vi "test Import Configuration File Max Channels.vi"(8 "error in":errorcluster, 11 "TestCase in":refnum<class "Import.lvclass">) -> (0 "error out":errorcluster, 3 "TestCase out":refnum<class "Import.lvclass">)   [LabVIEW 2020, in "Import.lvclass"]
uses:
  Import.lvclass
  Import.lvclass/Import.ctl
  C:/Program Files/National Instruments/LabVIEW 2026/vi.lib/addons/_JKI Toolkits/VI Tester/TestCase.llb/TestCase.lvclass
  C:/git/fmussi_niveristand-aim-arinc429-custom-device/Source/Custom Device Support/Tests/Unit/Import/Import.lvclass
  <vilib>/addons/_JKI Toolkits/VI Tester/TestCase.llb/TestCase.lvclass
  Import/ARINC 429 Import.lvlib
  <userlib>/_OpenG.lib/appcontrol/appcontrol.llb/openg_application_control.lvlib
  <vilib>/NI/VeriStand Custom Device Testing Tools/VeriStandTestUtilities/VeriStandTestUtilities.lvlib
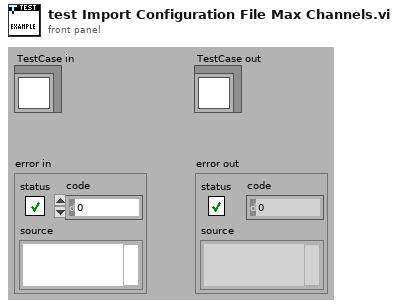
[diagram p1: front panel]
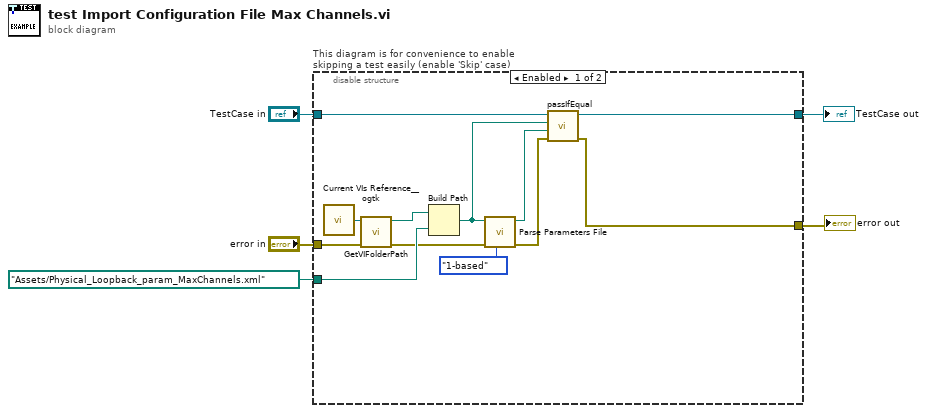
[diagram p0: block diagram]
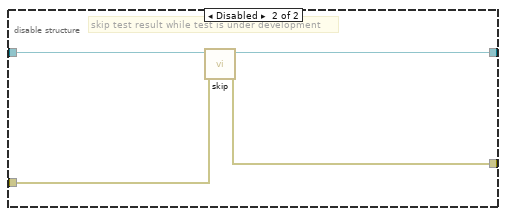
[diagram p2: hidden frame]
diagram:
  n1 = disable-structure "This diagram is for convenience to enable skipping a test easily (enable 'Skip' case)" shown="Enabled" {
    disable-tunnel: "TestCase in" -> [w17 w21]
    disable-tunnel: [w9 w19] -> w2
    disable-tunnel: [w10 w20] -> w4
    disable-tunnel: "error in" -> [w14 w18]
    disable-tunnel: path "Assets/Physical_Loopback_param_MaxChannels.xml" ("Absolute or Relative Path") -> [w13 _]
    frame Enabled {
      n2 = call <userlib>:"Current VIs Reference__ogtk.vi"() -> ("Current VI's reference"=w16:refnum<vi>)  [unwired: 5 in]
      n3 = call <vilib>:"GetVIFolderPath.vi"("error in (no error)"=w14, "VI Reference in"=w16) -> ("error out"=w11:errorcluster, "VI Folder Path out"=w15:path)  [unwired: 8 in]
      n4 = Build Path(base path=w15, name or relative path=w13) -> (appended path=w12:path)
      n5 = call "Parse Parameters File.vi"("ch indexing (0-based)"=enum16{"0-based", "1-based"}."1-based", "error in"=w11, "path to XML document"=w12) -> ("error out"=w8:errorcluster, "path to XML document out"=w7:path)  [unwired: 6 in, 1 out]
      n6 = call-dynamic "passIfEqual.vi"("error in (no error)"=w8, "y"=w7, "x"=w12, "TestCase in"=w17) -> ("error out"=w10:errorcluster, "TestCase out"=w9:refnum<class "Import.lvclass">)  [unwired: 6 in]
    }
    frame Disabled {
      # "skip test result while test is under development"
      n7 = call <vilib>:"skip.vi"("error in (no error)"=w18, "TestCase in"=w21) -> ("error out"=w20:errorcluster, "TestCase out"=w19:refnum<class "Import.lvclass">)  [unwired: 8 in]
    }
  }
  "error out" <- w4
  "TestCase out" <- w2
